vi "MotionProfileGenerator.vi"(1 "MotionProfileGeneratorParameters":T1={"Trajectory Point Interval (ms)"=10, "Maximum Travel Speed (units/s)"=0.0, "Velocity Ramp Time (ms)"=0.0, "Acceleration Ramp Time (ms)"=1.0} {"Acceleration Ramp Time (ms)" min=1.0; "Velocity Ramp Time (ms)" min=1.0; "Maximum Travel Speed (units/s)" min=0.0; "Trajectory Point Interval (ms)" items=["TrajectoryDuration_0ms"=0, "TrajectoryDuration_5ms"=5, "TrajectoryDuration_10ms"=10, "TrajectoryDuration_20ms"=20, "TrajectoryDuration_30ms"=30, "TrajectoryDuration_40ms"=40, "TrajectoryDuration_50ms"=50, "TrajectoryDuration_100ms"=100]}, 2 "Starting Position (units)":dbl, 3 "Travel Distance (units)":dbl) -> (0 "Trajectory Points":T3[](array[typedef]) {"Time (ms)" items=["TrajectoryDuration_0ms"=0, "TrajectoryDuration_5ms"=5, "TrajectoryDuration_10ms"=10, "TrajectoryDuration_20ms"=20, "TrajectoryDuration_30ms"=30, "TrajectoryDuration_40ms"=40, "TrajectoryDuration_50ms"=50, "TrajectoryDuration_100ms"=100]})   [LabVIEW 2017]
uses:
  TypeDefs/TrajectoryPoint.ctl
  <vilib>/Rock Robotics/WPI/ThirdParty/Phoenix-LabVIEW/Motor Controller/Controls/CTRE_Phoenix_MotorControl_TrajectoryPointTimeDur.ctl
  TypeDefs/MotionProfileGeneratorParams.ctl
panel:
  out "Input":bool
  out "T4":dbl
  out "fl2":dbl
  out "fl1":dbl
  out "n":dbl
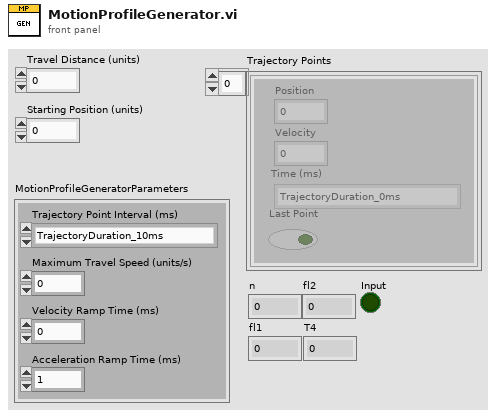
[diagram p1: front panel]
types:
  T1 = typedef "MotionProfileGeneratorParams.ctl" = cluster{"Trajectory Point Interval (ms)":T2, "Maximum Travel Speed (units/s)":dbl, "Velocity Ramp Time (ms)":dbl, "Acceleration Ramp Time (ms)":dbl}
  T2 = typedef "CTRE_Phoenix_MotorControl_TrajectoryPointTimeDur.ctl" = i32
  T3 = typedef "TrajectoryPoint.ctl" = cluster{"Position ":dbl, "Velocity ":dbl, "Time (ms)":T2, "Last Point":bool}
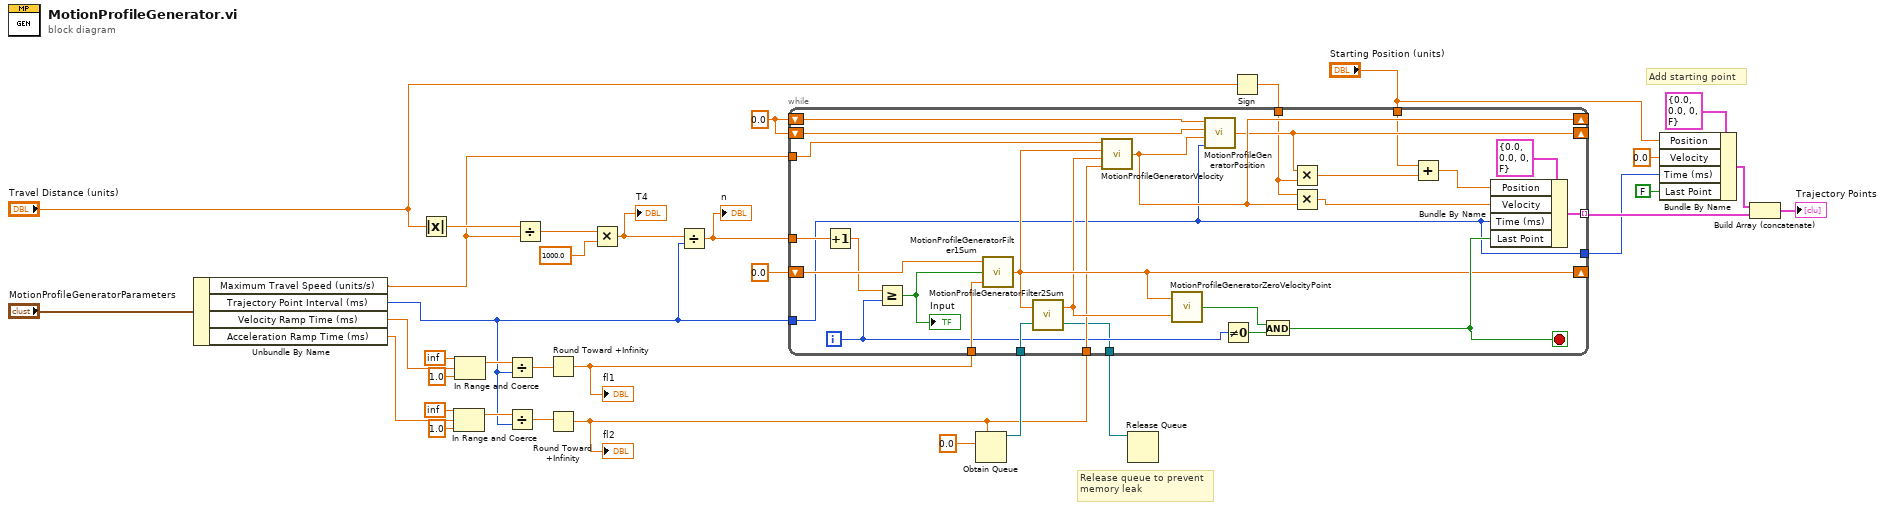
[diagram p0: block diagram]
diagram:
  w17 = 0.0
  # "Release queue to prevent\nmemory leak"
  # "Add starting point"
  n1 = Unbundle By Name("MotionProfileGeneratorParameters") -> ("Maximum Travel Speed (units/s)"=w1:dbl, "Trajectory Point Interval (ms)"=w13:T2, "Velocity Ramp Time (ms)"=w12:dbl, "Acceleration Ramp Time (ms)"=w11:dbl)
  n2 = Absolute Value(x="Travel Distance (units)") -> (abs(x)=w26:dbl)
  n3 = In Range and Coerce(upper limit=inf, x=w11, lower limit=1.0) -> (coerced(x)=w22:dbl)  [unwired: 1 out]
  n4 = In Range and Coerce(upper limit=inf, x=w12, lower limit=1.0) -> (coerced(x)=w23:dbl)  [unwired: 1 out]
  n5 = Divide(x=w23, y=w13) -> (x/y=w32:dbl)
  n6 = Divide(x=w22, y=w13) -> (x/y=w33:dbl)
  n7 = Divide(x=w26, y=w1) -> (x/y=w35:dbl)
  n8 = Round Toward +Infinity(x=w32) -> (ceil(x): smallest int >= x=w25:dbl)
  "fl1" <- w25
  n9 = Round Toward +Infinity(x=w33) -> (ceil(x): smallest int >= x=w24:dbl)
  "fl2" <- w24
  n10 = Multiply(x=w35, y=1000.0) -> (x*y=w31:dbl)
  "T4" <- w31
  n11 = Divide(x=w31, y=w13) -> (x/y=w30:dbl)
  "n" <- w30
  n12 = Obtain Queue(max queue size (-1, unlimited)=w24, element data type=0.0) -> (queue out=w27:refnum<queue>)  [unwired: 3 in, 2 out]
  n13 = Sign(1:"Travel Distance (units)") -> (0:w15:dbl)
  n14 = while {
    tunnel: w13 -> [w36]
    tunnel: w30 -> [w62]
    shift-right: [w51] -> _
    shift-left: 0.0 -> [w53]
    tunnel: w27 -> [w55]
    tunnel: [w59] -> w4 mode=indexing
    tunnel: w24 -> [w49]
    tunnel: w1 -> [w52]
    shift-right: [w44] -> _
    shift-left: w17 -> [w57]
    shift-right: [w42] -> _
    shift-left: w17 -> [w48]
    tunnel: w25 -> [w54]
    tunnel: w15 -> [w41]
    tunnel: [w38] -> w10
    tunnel: "Starting Position (units)" -> [w37]
    tunnel: [w36] -> w3
    i -> [w47]
    stop <- w58 stop-if-true
    n15 = Increment(x=w62) -> (x+1=w46:dbl)
    n16 = Greater Or Equal?(x=w46, y=w47) -> (x >= y?=w45:bool)
    "Input" <- w45
    n17 = call "MotionProfileGeneratorFilter1Sum.vi"("fl1"=w54, "Input"=w45, "Previous Filter1Sum"=w53) -> ("Filter1Sum"=w51:dbl)
    n18 = call "MotionProfileGeneratorFilter2Sum.vi"("Filter Queue"=w55, "Filter1Sum"=w51) -> ("queue out"=w38:refnum<queue>, "Filter2Sum"=w50:dbl)
    n19 = call "MotionProfileGeneratorVelocity.vi"("FL2"=w49, "filter2sum"=w50, "Filter1Sum"=w51, "Maximum Travel Speed (rps)"=w52) -> ("Velocity"=w44:dbl)
    n20 = call "MotionProfileGeneratorZeroVelocityPoint.vi"("Filter2Sum"=w50, "Filter1Sum"=w51) -> ("Zero Velocity"=w56:bool)
    n21 = call "MotionProfileGeneratorPosition.vi"("Trajectory Point Interval (ms)"=w36, "Velocity"=w44, "Previous Position"=w48, "Previous Velocity"=w57) -> ("Position"=w42:dbl)
    n22 = Not Equal To 0?(x=w47) -> (x != 0?=w61:bool)
    n23 = And(x=w56, y=w61) -> (x .and. y?=w58:bool)
    n24 = Multiply(x=w42, y=w41) -> (x*y=w40:dbl)
    n25 = Multiply(x=w41, y=w44) -> (x*y=w43:dbl)
    n26 = Add(x=w37, y=w40) -> (x+y=w39:dbl)
    n27 = Bundle By Name(cluster=T3 {"Position "=0.0, "Velocity "=0.0, "Time (ms)"=0, "Last Point"=FALSE} ("trajectory point"), "Position"=w39, "Velocity"=w43, "Time (ms)"=w36, "Last Point"=w58) -> (w59:T3)
  }
  n28 = Release Queue(queue=w10) -> ()  [unwired: 2 in, 3 out]
  n29 = Bundle By Name(cluster=T3 {"Position "=0.0, "Velocity "=0.0, "Time (ms)"=0, "Last Point"=FALSE} ("trajectory point"), "Position"="Starting Position (units)", "Velocity"=0.0, "Time (ms)"=w3, "Last Point"=FALSE) -> (w8:T3)
  n30 = Build Array (concatenate)(w8, w4) -> (→"Trajectory Points":T3[])
